vi "Create.vi"(7 "Direction":T1, 8 "error in (no error)":errorcluster, 9 "Custom Config Data":u8[](array[numeric]), 10 "Name":string, 11 "CIFFIFO in":refnum<class "CIF_CIPC_Fifo_U8.lvclass">) -> (0 "error out":errorcluster, 3 "CIFFIFO out":refnum<class "CIF_CIPC_Fifo_U8.lvclass">)   [LabVIEW 2021, in "CIF_CIPC_Fifo_U8.lvclass"]
uses:
  CIF_CIPC_Fifo_U8.lvclass
  <vilib>/CIF Foundation/CIF Channels Core/ChannelCommon/typedef/Direction.ctl
  C:/Program Files/National Instruments/LabVIEW 2021/vi.lib/CIF Foundation/CIF Channels Core/CIFChannels/CIFChannels.lvclass
  D:/dev/Packages/CIF_Channels_CIPC/src/CIPC_Channels/CIF_CIPC_Chan/CIF_CIPC_Chn.lvclass
  <vilib>/CIF Foundation/CIF Utilities/Statistics/I64/Stats_I64_CIF_U.lvclass/Stats_I64_CIF_U.ctl
  <vilib>/CIF Foundation/CIF Channels Core/ChannelCommon/typedef/Channel State.ctl
  <vilib>/CIF Foundation/CIF Channels Core/ChannelCommon/typedef/Disconnect Behavior.ctl
  <vilib>/CIF Foundation/CIF Channels Core/CIFChannels/CIFChannels.lvclass/CIFChannels.ctl
  <vilib>/CIF Foundation/CIF Channels Core/ChannelCommon/typedef/Channel Pattern.ctl
  CIF_CIPC_Chan/Typedef/Buffer Configuration Data.ctl
  <vilib>/CIF Foundation/CIF CIPC/TypeDefs/Backpressure References.ctl
  <vilib>/CIF Foundation/CIF CIPC/TypeDefs/Backpressure Names.ctl
  CIF_CIPC_Chan/CIF_CIPC_Chn.lvclass/CIF_CIPC_Chn.ctl
  CIF_CIPC_Fifo_U8.lvclass/CIF_CIPC_Fifo_U8.ctl
  35849dc3-58aa-4d75-b906-fe3df34869a7.vi
  <vilib>/CIF Foundation/CIF Channels Core/CIFChannels/Accessors/Write Pattern.vi
  CIF_CIPC_Chan/Accessors/Write Buffer Configuration.vi
  CIF_CIPC_Chan/Accessors/Write CIPC Channel.vi
  9be4d617-3037-4515-bcea-2a1e3727d04e.vi
  <vilib>/CIF Foundation/CIF Channels Core/CIFChannels/Accessors/Write Channel State.vi
  <vilib>/CIF Foundation/CIF Channels Core/CIFChannels/Accessors/Write Subscriber Count.vi
  <vilib>/CIF Foundation/CIF Channels Core/CIFChannels/Accessors/Write Channel Benchmark.vi
  <vilib>/CIF Foundation/CIF Channels Core/CIFChannels/Accessors/Write Flatten Benchmark.vi
  35849dc3-58aa-4d75-b906-fe3df34869a7.vi/bd07d5d9-1209-45ad-b636-9e9ab86132fb.vi
  <vilib>/CIF Foundation/CIF CIPC/SubVIs/Check Error.vi
  <vilib>/CIF Foundation/CIF CIPC/SubVIs/Add CIPC Error.vi
  <vilib>/CIF Foundation/CIF CIPC/SubVIs/Get dll Path.vi
  9be4d617-3037-4515-bcea-2a1e3727d04e.vi/49b3dd2d-4579-4089-b72e-3f0875c862f2.vi
  9be4d617-3037-4515-bcea-2a1e3727d04e.vi/1e2c93d0-55b0-4d6c-a9da-21395a664279.vi
  9be4d617-3037-4515-bcea-2a1e3727d04e.vi/7bb13226-97f3-4dcb-9346-06ec631a2876.vi
  9be4d617-3037-4515-bcea-2a1e3727d04e.vi/49b3dd2d-4579-4089-b72e-3f0875c862f2.vi/bd07d5d9-1209-45ad-b636-9e9ab86132fb.vi
  9be4d617-3037-4515-bcea-2a1e3727d04e.vi/1e2c93d0-55b0-4d6c-a9da-21395a664279.vi/49b3dd2d-4579-4089-b72e-3f0875c862f2.vi
  <vilib>/CIF Foundation/CIF CIPC/SubVIs/Notify Of New Write.vi
  <vilib>/CIF Foundation/CIF CIPC/SubVIs/Get Element Write Position.vi
  <vilib>/CIF Foundation/CIF CIPC/SubVIs/Get Element Description Variant.vi
  <vilib>/Utility/error.llb/Trim Whitespace.vi
  <vilib>/string/Create NI GUID.vi
  <vilib>/CIF Foundation/CIF CIPC/SubVIs/Check Error Core.vi
  <vilib>/CIF Foundation/CIF CIPC/SubVIs/Add CIPC Error Core.vi
  <vilib>/CIF Foundation/CIF CIPC/SubVIs/Get Backpressure Name.vi
  <vilib>/CIF Foundation/CIF CIPC/SubVIs/Get Element Info Variant.vi
  <vilib>/CIF Foundation/CIF Utilities/Statistics/I64/Stats_I64_CIF_U.lvclass
  <vilib>/CIF Foundation/CIF Channels Core/CIFChannels/CIFChannels.lvclass
  <vilib>/CIF Foundation/CIF Channels Core/ChannelCommon/ChannelCommon.lvlib
  <vilib>/CIF Foundation/CIF CIPC/CIF_NI_CIPC.lvlib
  CIF_CIPC_Chan/CIF_CIPC_Chn.lvclass
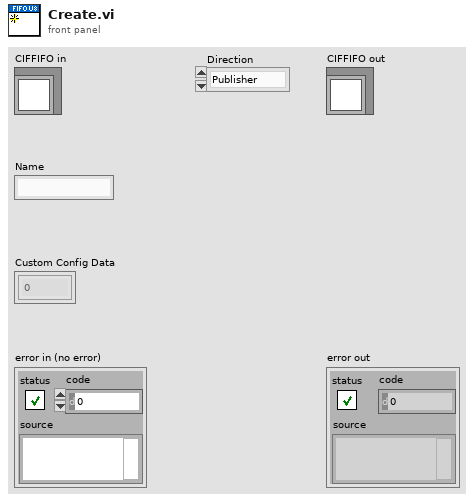
[diagram p1: front panel]
types:
  T1 = typedef "ChannelCommon.lvlib/Direction.ctl" = enum8{"Publisher", "Subscriber"}
  T2 = typedef "ChannelCommon.lvlib/Channel State.ctl" = enum8{"Creating", "Disconnected", "Connecting", "Connected", "Destroyed"}
  T3 = typedef "ChannelCommon.lvlib/Disconnect Behavior.ctl" = enum8{"Default value", "Last value", "Error with default"}
  T4 = typedef "ChannelCommon.lvlib/Channel Pattern.ctl" = enum8{"Unknown", "Tag", "FIFO", "MultiFIFO", "BackpressureFIFO"}
  T5 = typedef "CIF_CIPC_Chn.lvclass/Buffer Configuration Data.ctl" = cluster{"Total Size":u32, "Read Size":u32, "Read Offset":u32, "CIPC BP References":T6, "CIPC Backpressure Names":T7, "Override CIPC Name":string, "Encoder Data":string}
  T6 = typedef "CIF_NI_CIPC.lvlib/Backpressure References.ctl" = cluster{"CIPC Reference":u64, "CIPC BP Reference":u64}
  T7 = typedef "CIF_NI_CIPC.lvlib/Backpressure Names.ctl" = cluster{"CIPC Name":string, "CIPC BP Name":string}
  T8 = typedef "CIF_NI_CIPC.lvlib/Encoder Info.ctl" = cluster{"Name":string, "Version":i32, "Data":string}
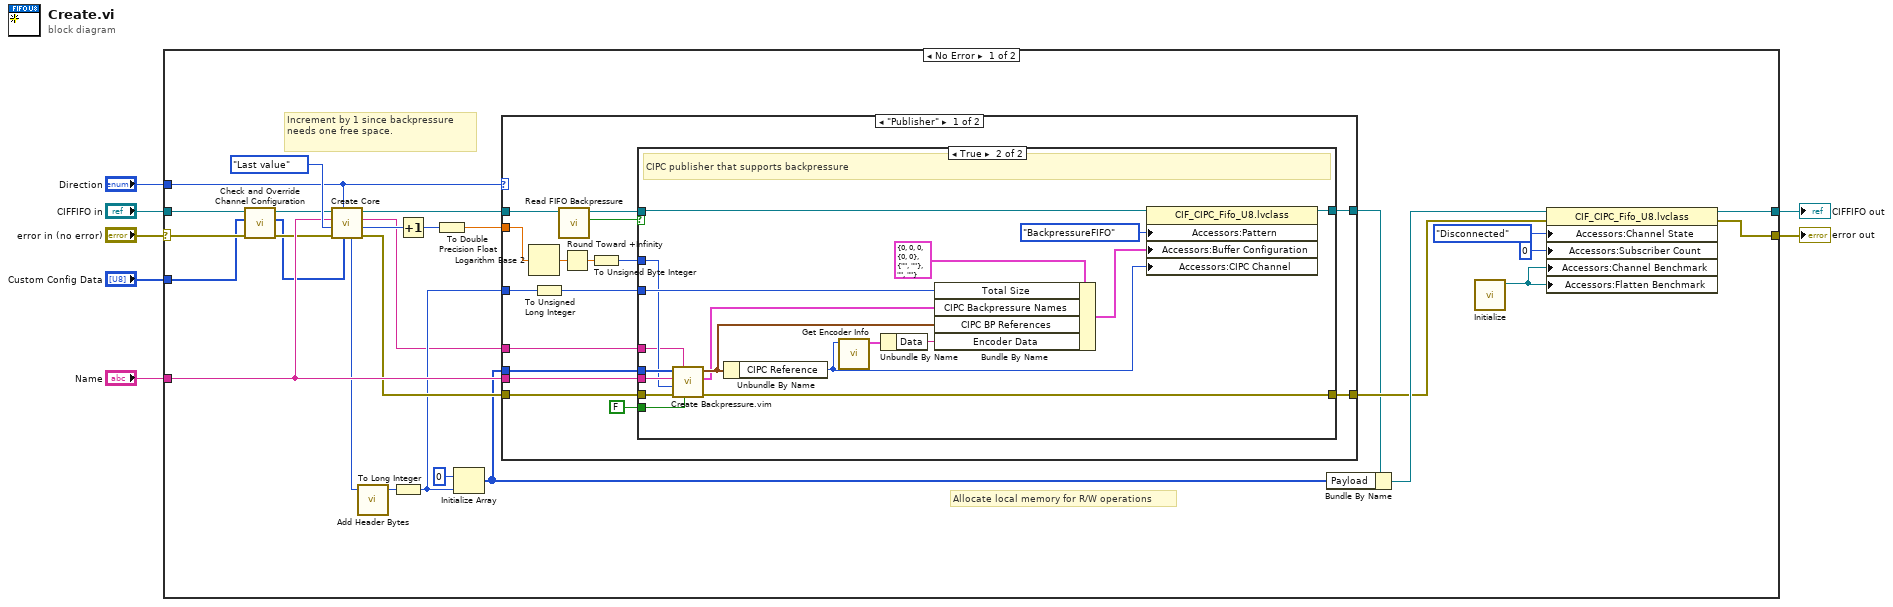
[diagram p0: block diagram]
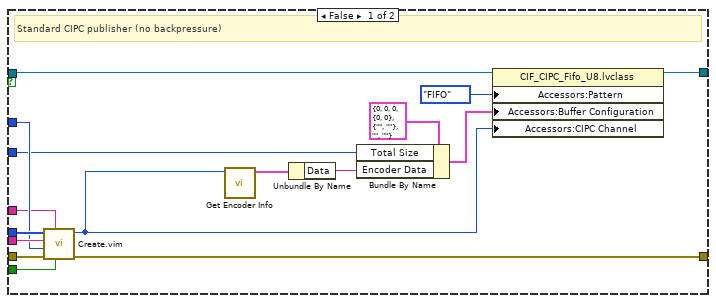
[diagram p2: hidden frame]
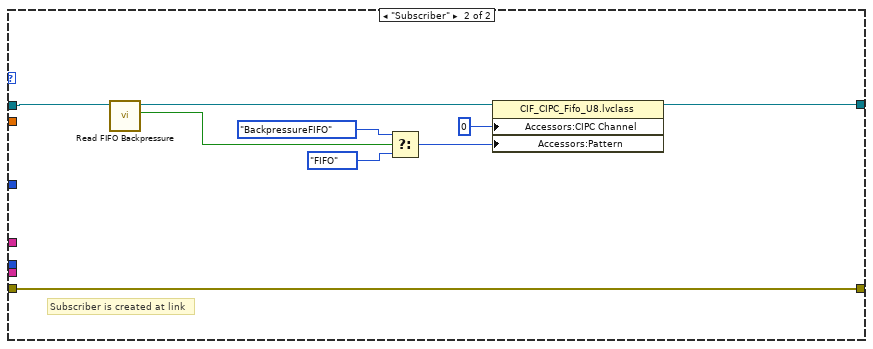
[diagram p3: hidden frame]
diagram:
  n1 = case shown="No Error" "error in (no error)" {
    selector: "error in (no error)" -> [w24 w96]
    tunnel: [w34 w96] -> w6
    tunnel: [w29 w95] -> w1
    tunnel: "CIFFIFO in" -> [w25 w95]
    tunnel: "Name" -> [w33 _]
    tunnel: "Direction" -> [w28 _]
    tunnel: "Custom Config Data" -> [w21 _]
    frame No Error {
      # "Increment by 1 since backpressure needs one free space."
      # "Allocate local memory for R/W operations"
      n2 = call-dynamic "Check and Override Channel Configuration.vi"("error in (no error)"=w24, "Custom Config Data in"=w21, "CIFFIFO in"=w25) -> ("error out"=w22:errorcluster, "Custom Config Data out"=w20:u8[], "CIFFIFO out"=w23:refnum<class "CIF_CIPC_Fifo_U8.lvclass">)  [unwired: 6 in]
      n3 = call <vilib>:"Create Core.vi"("Custom Config Data"=w20, "Direction"=w28, "error in (no error)"=w22, "Disconnect Behavior"=Disconnect_Behavior."Last value", "Name"=w33, "CIFChannels in"=w23) -> ("error out"=w32:errorcluster, "Messages"=w12:u64, "Channel Type"=w10:string, "CIFChannels out"=w16:refnum<class "CIF_CIPC_Fifo_U8.lvclass">, "Bytes/Msg"=w19:u64)  [unwired: 1 in]
      n4 = call <vilib>:"Add Header Bytes.vi"("Bytes/Msg"=w19) -> ("Bytes/Msg with header"=w15:u64)  [unwired: 3 in]
      n5 = To Long Integer(number=w15) -> (32bit integer=w14:i32)
      n6 = Increment(x=w12) -> (x+1=w11:u64)
      n7 = To Double Precision Float(number=w11) -> (double precision float=w17:dbl)
      n8 = Initialize Array(u8 0 ("Numeric"), w14) -> (w18:u8[])
      n9 = case shown="\"Publisher\"" w28 {
        tunnel: w33 -> [w48 _]
        tunnel: w32 -> [w50 w94]
        tunnel: [w51 w94] -> w30
        tunnel: w17 -> [w45 _]
        tunnel: w18 -> [w47 _]
        tunnel: w16 -> [w42 w91]
        tunnel: w14 -> [w39 _]
        tunnel: [w37 w93] -> w13
        tunnel: w10 -> [w36 _]
        frame "Publisher" {
          n10 = Logarithm Base 2(1:w45) -> (0:w46:dbl)
          n11 = To Unsigned Long Integer(number=w39) -> (unsigned 32bit integer=w38:u32)
          n12 = call <vilib>:"Read FIFO Backpressure.vi"("CIFChannels in"=w42) -> ("Backpressure"=w40:bool, "CIFChannels out"=w41:refnum<class "CIF_CIPC_Fifo_U8.lvclass">)  [unwired: 8 in, 1 out]
          n13 = Round Toward +Infinity(x=w46) -> (ceil(x): smallest int >= x=w44:dbl)
          n14 = To Unsigned Byte Integer(number=w44) -> (unsigned 8bit integer=w43:u8)
          n15 = case shown="True" w40 {
            tunnel: [w67 w75] -> w51
            tunnel: w50 -> [w66 w76]
            tunnel: FALSE ("Prepend Array Size") -> [w65 w79]
            tunnel: w48 -> [w64 w78]
            tunnel: w47 -> [w63 w80]
            tunnel: w43 -> [w62 w77]
            tunnel: w41 -> [w61 w85]
            tunnel: w38 -> [w59 w84]
            tunnel: [w55 w81] -> w37
            tunnel: w36 -> [w54 w72]
            frame False {
              # "Standard CIPC publisher (no backpressure)"
              n16 = call "Create.vim"("Prepend Array Size"=w65, "Description"=w54, "error in (no error)"=w66, "Buffer Size N (2^N)"=w62, "Name in"=w64, "Data Type"=w63) -> ("error out"=w67:errorcluster, "CIPC Reference"=w56:u64)  [unwired: 2 in, 2 out]
              n17 = call <vilib>:"Get Encoder Info.vi"("CIPC Reference"=w56) -> ("Encoder Info"=w58:T8)  [unwired: 9 in, 1 out]
              n18 = Unbundle By Name(w58) -> ("Data"=w57:string)
              n19 = Bundle By Name(cluster=T5 {"Total Size"=0, "Read Size"=0, "Read Offset"=0, "CIPC BP References"={"CIPC Reference"=0, "CIPC BP Reference"=0}, "CIPC Backpressure Names"={"CIPC Name"="", "CIPC BP Name"=""}, "Override CIPC Name"="", "Encoder Data"=""} ("Buffer Configuration"), "Total Size"=w59, "Encoder Data"=w57) -> (w53:T5)
              n20 = property class="CIF_CIPC_Fifo_U8.lvclass"(reference=w61, "Accessors:Pattern"=Channel_Pattern."FIFO" ("Pattern"), "Accessors:Buffer Configuration"=w53, "Accessors:CIPC Channel"=w56) -> (reference out=w55:refnum<class "CIF_CIPC_Fifo_U8.lvclass">)  [unwired: 1 in, 1 out]
            }
            frame True {
              # "CIPC publisher that supports backpressure"
              n21 = call "Create Backpressure.vim"("Prepend Array Size"=w79, "Description"=w72, "error in (no error)"=w76, "Buffer Size N (2^N)"=w77, "Name in"=w78, "Data Type"=w80) -> ("error out"=w75:errorcluster, "CIPC Backpressure Names"=w69:T7, "CIPC BP References"=w73:T6)  [unwired: 2 in, 1 out]
              n22 = Unbundle By Name(w73) -> ("CIPC Reference"=w74:u64)
              n23 = call <vilib>:"Get Encoder Info.vi"("CIPC Reference"=w74) -> ("Encoder Info"=w83:T8)  [unwired: 9 in, 1 out]
              n24 = Unbundle By Name(w83) -> ("Data"=w82:string)
              n25 = Bundle By Name(cluster=T5 {"Total Size"=0, "Read Size"=0, "Read Offset"=0, "CIPC BP References"={"CIPC Reference"=0, "CIPC BP Reference"=0}, "CIPC Backpressure Names"={"CIPC Name"="", "CIPC BP Name"=""}, "Override CIPC Name"="", "Encoder Data"=""} ("Buffer Configuration"), "Total Size"=w84, "CIPC Backpressure Names"=w69, "CIPC BP References"=w73, "Encoder Data"=w82) -> (w68:T5)
              n26 = property class="CIF_CIPC_Fifo_U8.lvclass"(reference=w85, "Accessors:Pattern"=Channel_Pattern."BackpressureFIFO" ("Pattern"), "Accessors:Buffer Configuration"=w68, "Accessors:CIPC Channel"=w74) -> (reference out=w81:refnum<class "CIF_CIPC_Fifo_U8.lvclass">)  [unwired: 1 in, 1 out]
            }
          }
        }
        frame "Subscriber" {
          # "Subscriber is created at link"
          n27 = call <vilib>:"Read FIFO Backpressure.vi"("CIFChannels in"=w91) -> ("Backpressure"=w89:bool, "CIFChannels out"=w90:refnum<class "CIF_CIPC_Fifo_U8.lvclass">)  [unwired: 8 in, 1 out]
          n28 = Select(t=Channel_Pattern."BackpressureFIFO" ("Pattern"), s=w89, f=Channel_Pattern."FIFO" ("Pattern")) -> (s? t:f=w86:T4)
          n29 = property class="CIF_CIPC_Fifo_U8.lvclass"(reference=w90, "Accessors:CIPC Channel"=u64 0 ("CIPC Channel"), "Accessors:Pattern"=w86) -> (reference out=w93:refnum<class "CIF_CIPC_Fifo_U8.lvclass">)  [unwired: 1 in, 1 out]
        }
      }
      n30 = Bundle By Name(cluster=w13, "Payload"=w18) -> (w31:refnum<class "CIF_CIPC_Fifo_U8.lvclass">)
      n31 = call <vilib>:"Initialize.vi"() -> ("Stats_I64_CIF_U out"=w26:refnum<class "Stats_I64_CIF_U.lvclass">)  [unwired: 10 in, 1 out]
      n32 = property class="CIF_CIPC_Fifo_U8.lvclass"(reference=w31, error in=w30, "Accessors:Channel State"=Channel_State."Disconnected" ("Channel State"), "Accessors:Subscriber Count"=u32 0 ("Subscriber Count"), "Accessors:Channel Benchmark"=w26, "Accessors:Flatten Benchmark"=w26) -> (reference out=w29:refnum<class "CIF_CIPC_Fifo_U8.lvclass">, error out=w34:errorcluster)
    }
    frame Error {
    }
  }
  "error out" <- w6
  "CIFFIFO out" <- w1
